vi "[ce] ODE R-K Solver of dX(t)_dt=F(t) particular case.vi"(4 "parameters":cluster{"name":string, "value":dbl}[](array[cluster]) {"value" format="%.2f"}, 6 "time":string="t", 7 "h (step rate)":dbl=0.1 format="%.4f", 8 "error in":errorcluster, 9 "equation info":cluster{"formula":string, "init value":dbl} {"init value" format="%.2f"}, 10 "time end":dbl=1.0 format="%.2f", 11 "time start":dbl format="%.2f") -> (0 "error out":errorcluster, 1 "ticks":u32, 2 "X Values (solution)":dbl[](array[numeric]) format="%.2f", 3 "Times":dbl[](array[numeric]) format="%.2f")   [LabVIEW 2021]
doc: "This VI uses Runge Kutta method to solve particular case of ordinary differential equation when solution depends only on a time variable:\n dX(t)/dt = F(t) , X(0) = X0\nIn addition, the VI allows specifying additional parameters and evaluating them in formula.\n\nIn this particular case the Runge Kutta method can be written as it's shown below\n k1 = F(t)\n k2 = F(t+h/2)\n k3 = F(t+h/2)\n k4 = F(t+h)\n x = x0 + h * (k1/6 + k2/3 + k3/3 + k4/6)\n\nafter a few simple transformations it can be simplified\n k1 = F(t)\n k23 = 4*F(t+h/2)\n k4 = F(t+h)\n x = x0 + h * (k1 + k23 + k4)/6\n\nThe VI uses this method and polymorphism feature of CalcExpress to solve the such equations very fast.\n\n::: CalcExpress Toolkit :::\nCopyright (c) 2000-2026 Konstantin Shifershteyn. All rights reserved."
panel:
  in  "info":string="This VI uses Runge Kutta method to solve particular case of ordinary differential equation when solution depends only on a time variable:\n  dX(t)/dt = F(t) ,  X(0) = X0\n\nIn this particular case the Runge Kutta method can be rewritten as shown below\n  k1 = F(t)\n  k2 = F(t+h/2)\n  k3 = F(t+h/2)\n  k4 = F(t+h)\n  x = x0 + h * (k1/6 + k2/3 + k3/3 + k4/6)\n\nafter a few simple transformations it can be simplified as shown below\n  k1   = F(t)\n  k23 = 4*F(t+h/2)\n  k4   = F(t+h)\n  x = x0 + h * (k1 + k23 + k4)/6\n\nThe VI uses this method to solve the such differential equations. Due to CalcExpress capability to make calculation with arrays the VI can determine the solution very fast.\n\nThis VI is used, for instance, to compute integral of f(x) functions. See [ce] Integration.vi\n\nExample:\n time start: 0.0\n time end:  10.0\n h:     0.1\n time: t\n equation info.formula:    sin(2*t)*exp(-t/3)\n equation info.init value: 0.0"
  # "dX(t)/dt = F(t) , X(0) = X0"
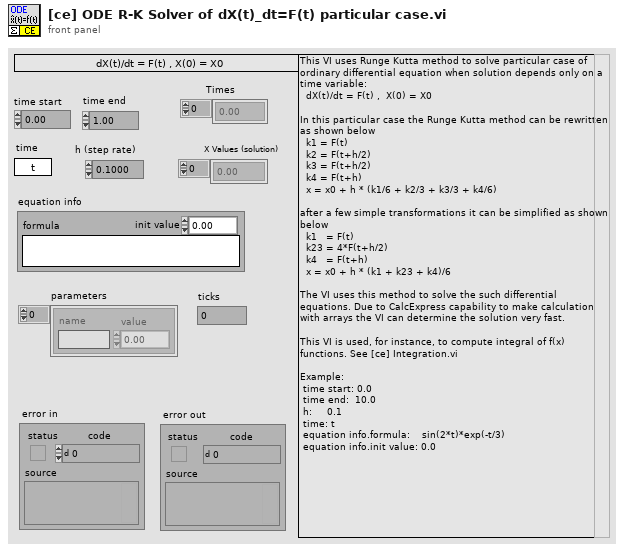
[diagram p1: front panel]
types:
  T1 = typedef "VarMan Variable Context Handle.ctl" = i32
  T2 = enum16{"create", "destroy", "set value", "get value"}
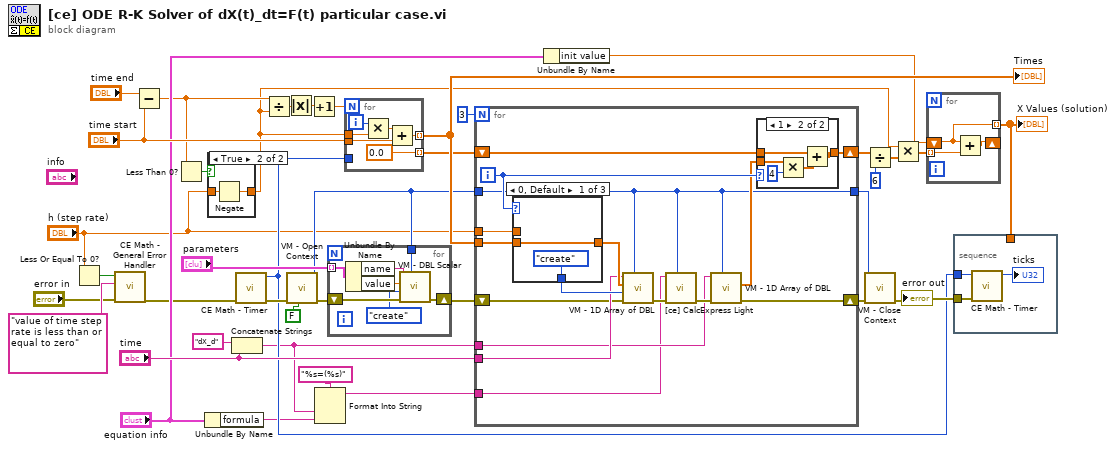
[diagram p0: block diagram]
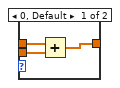
[diagram p3: hidden frame]
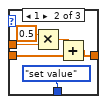
[diagram p4: hidden frame]
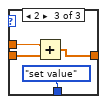
[diagram p5: hidden frame]
diagram:
  n1 = Less Or Equal To 0?(x="h (step rate)") -> (x <= 0?=w6:bool)
  n2 = call "CE Math - General Error Handler.vi"("error before"="error in", "message"="value of time step rate is less than or equal to zero", "error? (T)"=w6) -> ("error out"=w5:errorcluster)  [unwired: 5 in, 1 out]
  n3 = Subtract(x="time end", y="time start") -> (x-y=w9:dbl)
  n4 = Less Than 0?(x=w9) -> (x < 0?=w7:bool)
  n5 = Unbundle By Name("equation info") -> ("formula"=w12:string)
  n6 = case shown="True" w7 {
    tunnel: [w40 w41] -> w8
    tunnel: "h (step rate)" -> [w40 w42]
    frame False {
    }
    frame True {
      n7 = Negate(x=w42) -> (-x=w41:dbl)
    }
  }
  n8 = Concatenate Strings("dX_d" ("Substring"), "time") -> (w11:string)
  n9 = call "CE Math - Timer.vi"("error in (no error)"=w5) -> ("error out"=w27:errorcluster, "ticks out"=w14:u32)  [unwired: 7 in]
  n10 = Divide(x=w9, y=w8) -> (x/y=w38:dbl)
  n11 = Absolute Value(x=w38) -> (abs(x)=w33:dbl)
  n12 = call "VM - Open Context.vi"("close loose contexts (F)"=FALSE ("close loose contexts (T)"), "error in"=w27) -> ("error out"=w17:errorcluster, "VC Handle out"=w15:T1)  [unwired: 7 in, 1 out]
  n13 = Increment(x=w33) -> (x+1=w22:dbl)
  n14 = Format Into String(format string="%s=(%s)" ("Format String"), w11, w12) -> (resulting string=w10:string)  [unwired: 2 in, 1 out]
  n15 = for {
    shift-right: [w44] -> w16
    shift-left: w17 -> [w49]
    tunnel: w15 -> [w45]
    tunnel: "parameters" -> [w43] mode=indexing
    n16 = Unbundle By Name(w43) -> ("name"=w46:string, "value"=w47:dbl)
    n17 = call "VM - DBL Scalar.vi"("VC Handle"=w45, "error in"=w49, "cmd"=T2."create", "value in"=w47, "name_spec"=w46) -> ("error out"=w44:errorcluster)  [unwired: 1 in, 5 out]
  }
  n18 = for {
    N: w22 -> [_]
    tunnel: "time start" -> [w51]
    tunnel: w8 -> [w53]
    tunnel: [w55] -> w30 mode=indexing
    tunnel: [0.0 ("Element Data")] -> w19 mode=indexing
    tunnel: w14 -> [_]
    i -> [w52]
    n19 = Multiply(x=w52, y=w53) -> (x*y=w50:dbl)
    n20 = Add(x=w50, y=w51) -> (x+y=w55:dbl)
  }
  "Times" <- w30
  n21 = for {
    N: 3 -> [_]
    tunnel: w30 -> [w68]
    tunnel: "h (step rate)" -> [w67]
    tunnel: "time" -> [w65]
    tunnel: w11 -> [w64]
    tunnel: w10 -> [w63]
    shift-right: [w61] -> w32
    shift-left: w19 -> [w59]
    shift-right: [w57] -> w29
    shift-left: w16 -> [w58]
    tunnel: w15 -> [w56]
    tunnel: [w56] -> w28
    i -> [w62]
    n22 = case shown="0, Default" w62 {
      tunnel: [w81 w87 w89] -> w69
      tunnel: w68 -> [w81 w86 w91]
      tunnel: w67 -> [_ w84 w90]
      tunnel: [T2."create" ("cmd") T2."set value" ("cmd") T2."set value" ("cmd")] -> w66
      frame 0, Default {
      }
      frame 1 {
        n23 = Multiply(x=0.5 ("y"), y=w84) -> (x*y=w83:dbl)
        n24 = Add(x=w83, y=w86) -> (x+y=w87:dbl[])
      }
      frame 2 {
        n25 = Add(x=w90, y=w91) -> (x+y=w89:dbl[])
      }
    }
    n26 = call "VM - 1D Array of DBL.vi"("VC Handle"=w56, "error in"=w58, "cmd"=w66, "value in"=w69, "name_spec"=w65) -> ("error out"=w71:errorcluster)  [unwired: 1 in, 5 out]
    n27 = call "[ce] CalcExpress Light.vi"("VC Handle"=w56, "error in"=w71, "expression"=w63) -> ("error out"=w70:errorcluster)  [unwired: 6 in, 2 out]
    n28 = call "VM - 1D Array of DBL.vi"("VC Handle"=w56, "error in"=w70, "name_spec"=w64) -> ("error out"=w57:errorcluster, "value out"=w60:dbl[])  [unwired: 3 in, 4 out]
    n29 = case shown="1" w62 {
      tunnel: [w74 w79] -> w61
      tunnel: w60 -> [w72 w78]
      tunnel: w59 -> [w73 w76]
      frame 0, Default {
        n30 = Add(x=w73, y=w72) -> (x+y=w74:dbl[])
      }
      frame 1 {
        n31 = Multiply(x=w78, y=4) -> (x*y=w75:dbl[])
        n32 = Add(x=w76, y=w75) -> (x+y=w79:dbl[])
      }
    }
  }
  n33 = Unbundle By Name("equation info") -> ("init value"=w23:dbl)
  n34 = Divide(x=w32, y=6) -> (x/y=w20:dbl[])
  n35 = call "VM - Close Context.vi"("error in"=w29, "VC Handle"=w28) -> ("error out"=w26:errorcluster)  [unwired: 8 in, 1 out]
  "error out" <- w26
  n36 = Multiply(x=w8, y=w20) -> (x*y=w24:dbl[])
  n37 = for {
    shift-right: [w94] -> _
    shift-left: w23 -> [w93]
    tunnel: w24 -> [w92] mode=indexing
    tunnel: [w93] -> w21 mode=indexing
    n38 = Add(x=w93, y=w92) -> (x+y=w94:dbl)
  }
  "X Values (solution)" <- w21
  n39 = stacked-sequence {
    tunnel: w26 -> [w97]
    tunnel: w14 -> [w96]
    tunnel: w21 -> [_]
    frame #0 {
      n40 = call "CE Math - Timer.vi"("error in (no error)"=w97, "ticks in"=w96) -> ("ticks out"=→"ticks":u32)  [unwired: 6 in, 1 out]
    }
  }
